vi "Keep Latest Temperatures.vi"(0 "lines":string[](array[string]), 5 "buffer size":i32=3, 11 "error in":errorcluster) -> (4 "latest temperatures":dbl[](array[numeric]), 6 "dropped count":i32, 15 "error out":errorcluster)   [LabVIEW 2026]
doc: "Extracts a temperature from every line with the regular expression T=([0-9.]+)C (Match Regular Expression, first capture group) and keeps only the last buffer size values in a size-limited queue fed by Lossy Enqueue Element. Lines that do not match are skipped. Returns the kept temperatures oldest first and how many were pushed out (overflow? of Lossy Enqueue Element). The queue is released at the end. An incoming error skips the work and is passed through. A buffer size below 1 makes Obtain Queue report an error."
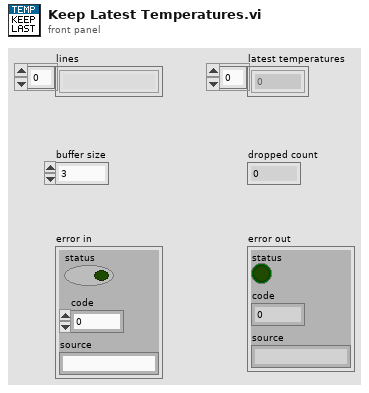
[diagram p1: front panel]
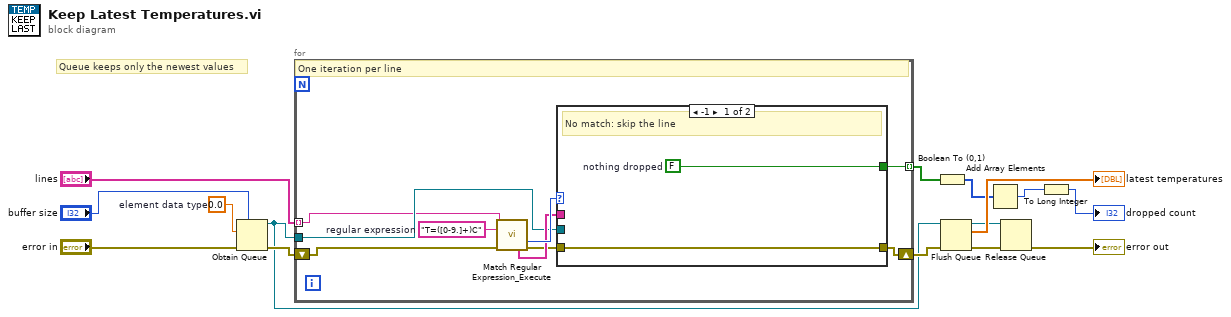
[diagram p0: block diagram]
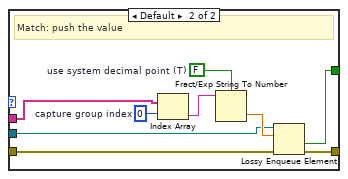
[diagram p2: hidden frame]
diagram:
  w4 = 0.0  # element data type
  # "Queue keeps only the newest values"
  n1 = Obtain Queue(max queue size (-1, unlimited)="buffer size", element data type=w4, error in (no error)="error in") -> (queue out=w5:refnum<queue>, error out=w6:errorcluster)  [unwired: 2 in, 1 out]
  n2 = for {
    tunnel: "lines" -> [w16] mode=indexing
    tunnel: w5 -> [w17]
    shift-right: [w19] -> w7
    shift-left: w6 -> [w18]
    tunnel: [w24] -> w8 mode=indexing
    w20 = "T=([0-9.]+)C"  # regular expression
    # "One iteration per line"
    n3 = call <vilib>:"Match Regular Expression_Execute.vi"("input string"=w16, "regular expression"=w20, "error in (no error)"=w18) -> ("whole match offset"=w23:i32, "matched substrings"=w22:string[], "error out"=w21:errorcluster)  [unwired: 7 in, 3 out]
    n4 = case shown="-1" w23 {
      tunnel: [w26 w34] -> w24
      tunnel: w17 -> [_ w27]
      tunnel: w21 -> [w25 w28]
      tunnel: w22 -> [_ w29]
      tunnel: [w25 w35] -> w19
      frame -1 {
        w26 = FALSE  # nothing dropped
        # "No match: skip the line"
      }
      frame Default {
        w32 = FALSE  # use system decimal point (T)
        w30 = 0  # capture group index
        # "Match: push the value"
        n5 = Index Array(array=w29, index=w30) -> (element=w31:string)
        n6 = Fract/Exp String To Number(use system decimal point (T)=w32, string=w31) -> (number=w33:dbl)  [unwired: 2 in, 1 out]
        n7 = Lossy Enqueue Element(queue=w27, element=w33, error in (no error)=w28) -> (overflow?=w34:bool, error out=w35:errorcluster)  [unwired: 2 out]
      }
    }
  }
  n8 = Boolean To (0,1)(Boolean=w8) -> (0, 1=w9:i16[])
  n9 = Flush Queue(queue=w5, error in (no error)=w7) -> (queue out=w12:refnum<queue>, remaining elements=→"latest temperatures":dbl[], error out=w14:errorcluster)
  n10 = Add Array Elements(numeric array=w9) -> (sum=w10:i16)
  n11 = Release Queue(queue=w12, error in (no error)=w14) -> (error out=→"error out":errorcluster)  [unwired: 1 in, 2 out]
  n12 = To Long Integer(number=w10) -> (32bit integer=→"dropped count":i32)
